vi "initModelv2.vi"(8 "error in (no error)":errorcluster, 10 "initModelv2Params":T1={"modelH"=736, "modelW"=1280, "frameH"=1280, "frameW"=720, "batchSize"=1, "conf"=0.6, "iou"=0.55}, 11 "dl in":refnum<class "dl.lvclass">) -> (0 "error out":errorcluster, 3 "dl out":refnum<class "dl.lvclass">)   [LabVIEW 2025, in "dl.lvlib" / "dl.lvclass"]
uses:
  dl.lvclass
  dl.lvclass/dl.ctl
  initModelv2Params.ctl
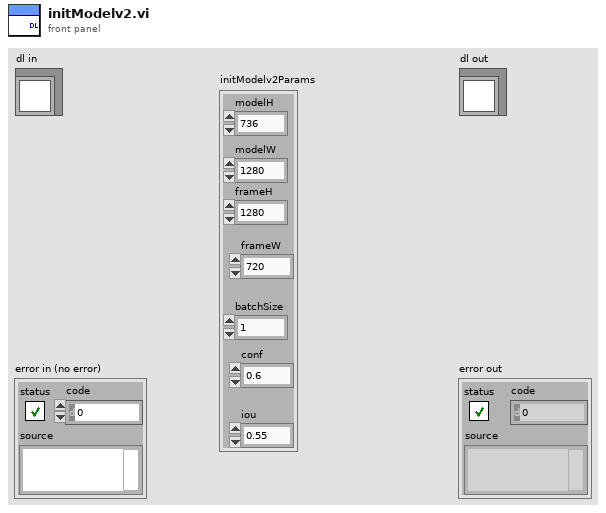
[diagram p1: front panel]
types:
  T1 = typedef "dl.lvlib/dl.lvclass/initModelv2Params.ctl" = cluster{"modelH":i32, "modelW":i32, "frameH":i32, "frameW":i32, "batchSize":i32, "conf":sgl, "iou":sgl}
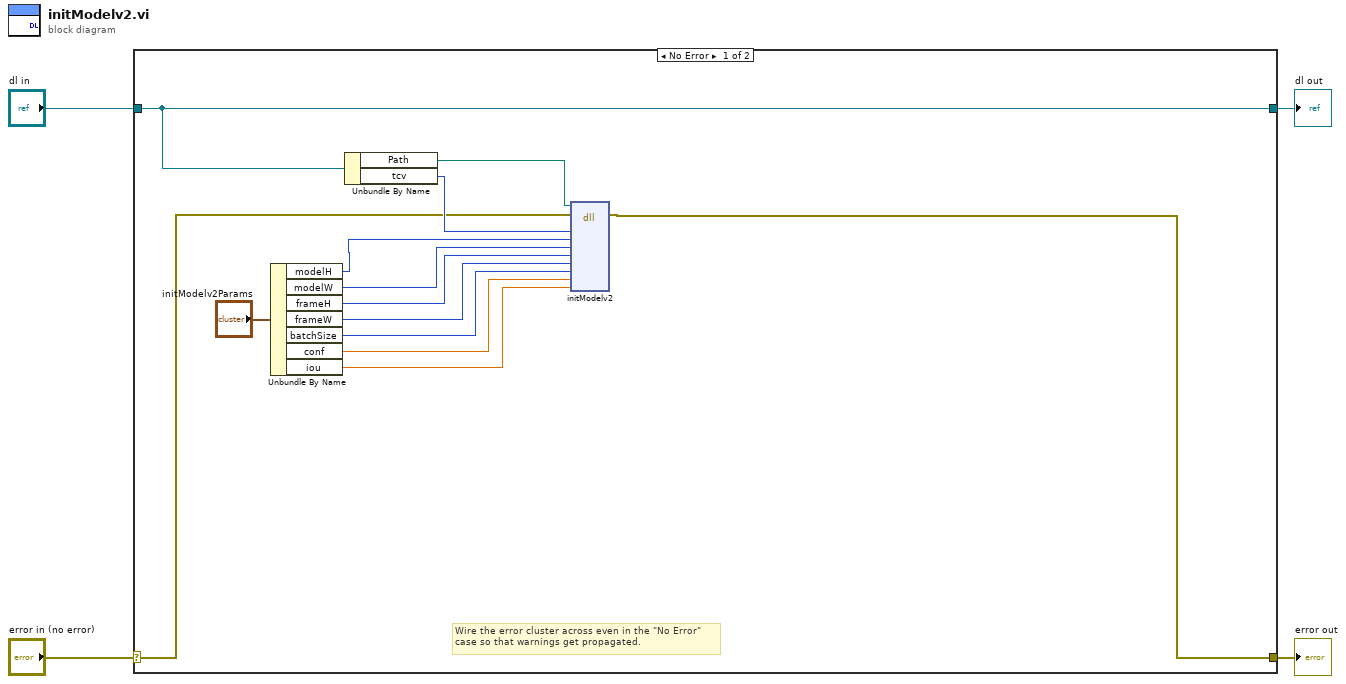
[diagram p0: block diagram]
diagram:
  n1 = case shown="No Error" "error in (no error)" {
    selector: "error in (no error)" -> [w14 w19]
    tunnel: [w13 w19] -> w3
    tunnel: [w17 w18] -> w1
    tunnel: "dl in" -> [w17 w18]
    frame No Error {
      # "Wire the error cluster across even in the \"No Error\"\ncase so that warnings get propagated."
      n2 = Unbundle By Name("initModelv2Params") -> ("modelH"=w11:i32, "modelW"=w10:i32, "frameH"=w9:i32, "frameW"=w8:i32, "batchSize"=w7:i32, "conf"=w6:sgl, "iou"=w5:sgl)
      n3 = Unbundle By Name(w17) -> ("Path"=w16:path, "tcv"=w15:u64)
      n4 = dll-call lib="C:/Program Files/ADS/Resources/TCV_Lib.dll" fn="initModelv2"(path in=w16, error in=w14, "tcv"=w15, "modelH"=w11, "modelW"=w10, "frameH"=w9, "frameW"=w8, "batchSize"=w7, "conf"=w6, "iou"=w5) -> (error out=w13:errorcluster)  [unwired: 10 in, 1 out]
    }
    frame Error {
    }
  }
  "error out" <- w3
  "dl out" <- w1
